vi "ECS - System - User Interface Calpoints.vi"   [LabVIEW 2015, in "ECS-RT.lvlib"]
uses:
  ECS-RT.lvlib
  Globals/Calpoint IDs.vi
  <vilib>/addons/Software Calibration Management/_CalPointResources/scm32.dll
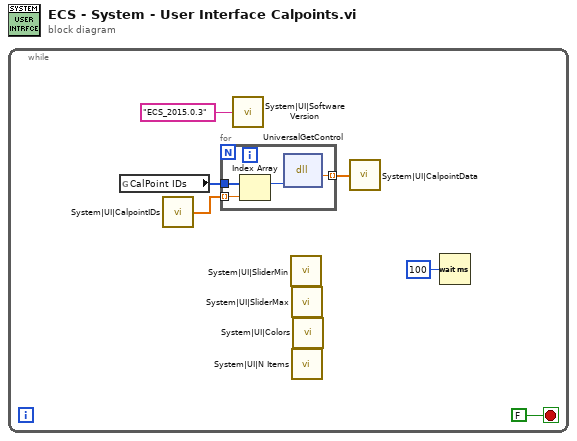
[diagram p0: block diagram]
diagram:
  n1 = while {
    stop <- FALSE stop-if-true
    n2 = global read "Calpoint IDs.vi" "CalPoint IDs"() -> (w6:i32[])
    n3 = call "System|UI|CalpointIDs"() -> ("Value"=w5:sgl[])
    n4 = for {
      tunnel: w6 -> [w10]
      tunnel: [w9] -> w4 mode=indexing
      tunnel: w5 -> [w7] mode=indexing
      n5 = Index Array(array=w10, index=w7) -> (element=w8:i32)
      n6 = dll-call lib="C:/Program Files (x86)/National Instruments/LabVIEW 2015/vi.lib/addons/Software Calibration Management/_CalPointResources/scm*.*" fn="UniversalGetControl"("ID"=w8) -> ("return type"=w9:sgl)  [unwired: 4 in, 2 out]
    }
    n7 = call "System|UI|Software Version"("Value"="ECS_2015.0.3") -> ()
    n8 = call "System|UI|SliderMin"() -> ()  [unwired: 1 out]
    n9 = call "System|UI|SliderMax"() -> ()  [unwired: 1 out]
    n10 = call "System|UI|N Items"() -> ()  [unwired: 1 out]
    n11 = call "System|UI|Colors"() -> ()  [unwired: 1 out]
    n12 = call "System|UI|CalpointData"("Value"=w4) -> ()
    n13 = Wait (ms)(milliseconds to wait=u32 100) -> ()  [unwired: 1 out]
  }
